vi "GetConfigurationType.vi"(8 "error in (no error)":errorcluster, 11 "object in":refnum<class "Channel.lvclass">) -> (0 "error out":errorcluster, 2 "Configuration":refnum<class "Configuration.lvclass">, 3 "object out":refnum<class "Channel.lvclass">)   [LabVIEW 2021, in "Channel.lvlib" / "Channel.lvclass"]
doc: "Gets the Default Value of the Configuration"
uses:
  Channel.lvclass
  Configuration_class/Configuration.lvclass
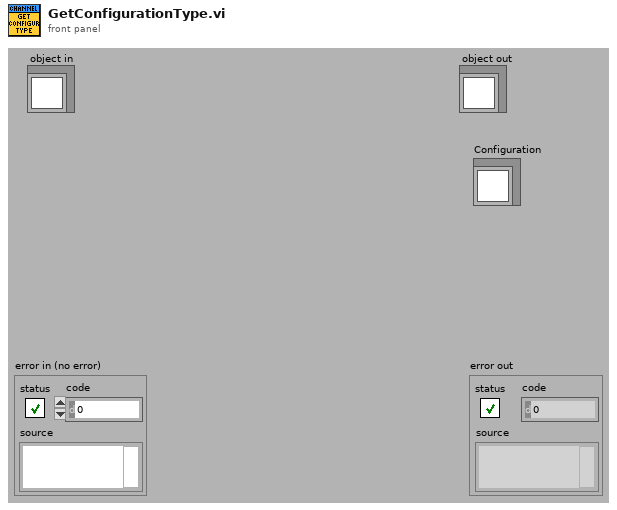
[diagram p1: front panel]
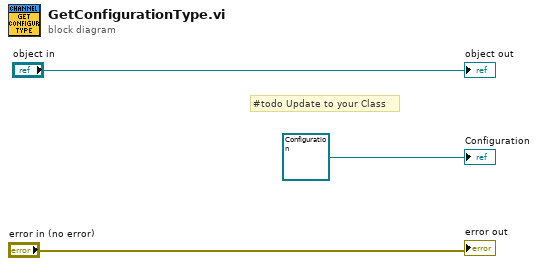
[diagram p0: block diagram]
diagram:
  # "#todo Update to your Class"
  "error out" <- "error in (no error)"
  "object out" <- "object in"
  "Configuration" <- refnum<class "Configuration.lvclass"> refnum ("Configuration")
